vi "Measurement UI.vi"() -> ()   [LabVIEW 2025, in "CAN-LIN Raw Bus Capture UI.lvlib"]
uses:
  CAN-LIN Raw Bus Capture UI.lvlib
  Toggle.ctl
  <vilib>/gRPC/LabVIEW gRPC Library/Shared/grpcId.ctl
  <vilib>/Utility/error.llb/whitespace.ctl
  <vilib>/Utility/error.llb/Trim Whitespace One-Sided.vi
  Get Status.vi
  Create Buffer.vi
  Flush Table.vi
  Destroy Table Buffer.vi
  OOB gRPC Client/OOB gRPC Client.lvlib
  <vilib>/gRPC/LabVIEW gRPC Library/grpc-lvsupport-release.lvlib
panel:
  out "New root item?":bool
  in  "Tree Data":string[][](array[string])
  in  "Mapping done?":bool
  in  "Table map":map{string, i32}(c390)
  in  "XNET Sessions map":map{u32, refnum<k21>}(c390)
  in  "Tags map":map{string, bool}(c390)
  out "Valid DBC file?":bool
  out "Signals in DBC":i32
  out "Frames in DBC":i32
  in  "Frames Map":map{u32, refnum<k21>}(c390)
  in  "Signals Map":map{u32, refnum<k21>[]}(c390)
  in  "Tree and Table":enum32{"Trace window", "Signal table"}(tab)
  out "Frames":string(tree)
  out "Signals":string[][](table)
  in  "HELP":bool
  out "IsRestarting?":bool
  out "Table Buffer":i32
  out "Error (Logic)":string
  out "Status Message":string
  in  "SAVE FORMAT":u16(ring) items=["TDMS", "CSV"]
  out "Connection":bool
  in  "Clear Trace":bool
  in  "Bus Type":string="CAN"
  in  "Lin Interface":string
  in  "Can Interface":string
  in  "PauseResume":bool
  in  "Path":path
  in  "Save":bool
  in  "Filter":string
  in  "SortByID":bool
  out "Status":string
  in  "SETTINGS":enum32{"CAN", "LIN"}(tab)
  in  "Run Mode":enum32{"Normal", "Subordinate"}(ring)
  in  "IO Mode":enum32{"CAN", "CAN FD", "CAN FD + BRS"}(ring)
  in  "FD ISO Mode":enum32{"ISO", "Non ISO", "Legacy ISO"}(ring)
  in  "Baudrate":u32=125000
  in  "FD Baudrate":u32=1000000
  in  "Termination CAN":T1
  in  "INTERFACE NAME CAN":refnum<k21>
  in  "DBC path":path
  in  "Termination LIN":T1
  in  "INTERFACE NAME LIN":refnum<k21>
  out "Buffer Size":i32
  out "OOB gRPC Port":i32
  # "CONFIGURATION"
  # "CONTROL"
  # "DBC INFORMATION"
  # "STATUS"
  # "CAN Settings"
  # "LIN Settings"
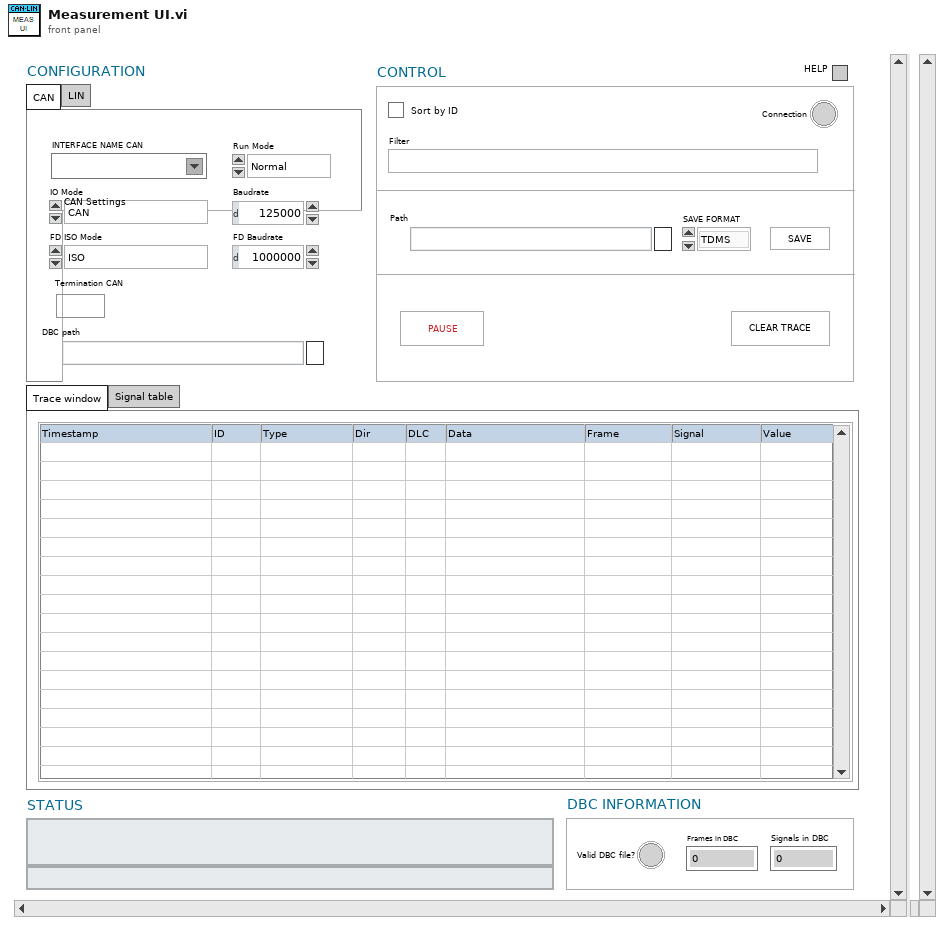
[diagram p1: front panel]
types:
  T1 = typedef "Toggle.ctl" = bool
  T2 = typedef "grpc-lvsupport-release.lvlib/grpcId.ctl" = u64
  T3 = cluster{"Tree and Table":refnum<vi>, "New root item?":refnum<vi>, "Tree Data":refnum<vi>, "Mapping done?":refnum<vi>, "Table map":refnum<vi>, "Tags map":refnum<vi>, "XNET Sessions map":refnum<vi>, "Signals":refnum<vi>, "PauseResume":refnum<vi>, "Clear Trace":refnum<vi>, "Path":refnum<vi>, "SAVE FORMAT":refnum<vi>, "Save":refnum<vi>, "Bus Type":refnum<vi>, "Filter":refnum<vi>, "SortByID":refnum<vi>, "Status Message":refnum<vi>, "Frames":refnum<vi>, "DBC path":refnum<vi>, "Signals Map":refnum<vi>, "Frames Map":refnum<vi>, "Frames in DBC":refnum<vi>, "Signals in DBC":refnum<vi>, "Valid DBC file?":refnum<vi>}
  T4 = typedef "whitespace.ctl" = u16
  T5 = enum32{"Page Enabled", "Page Disabled", "Page Disabled & Grayed"}
  T6 = enum8{"Enabled", "Disabled", "Disabled and Grayed Out"}
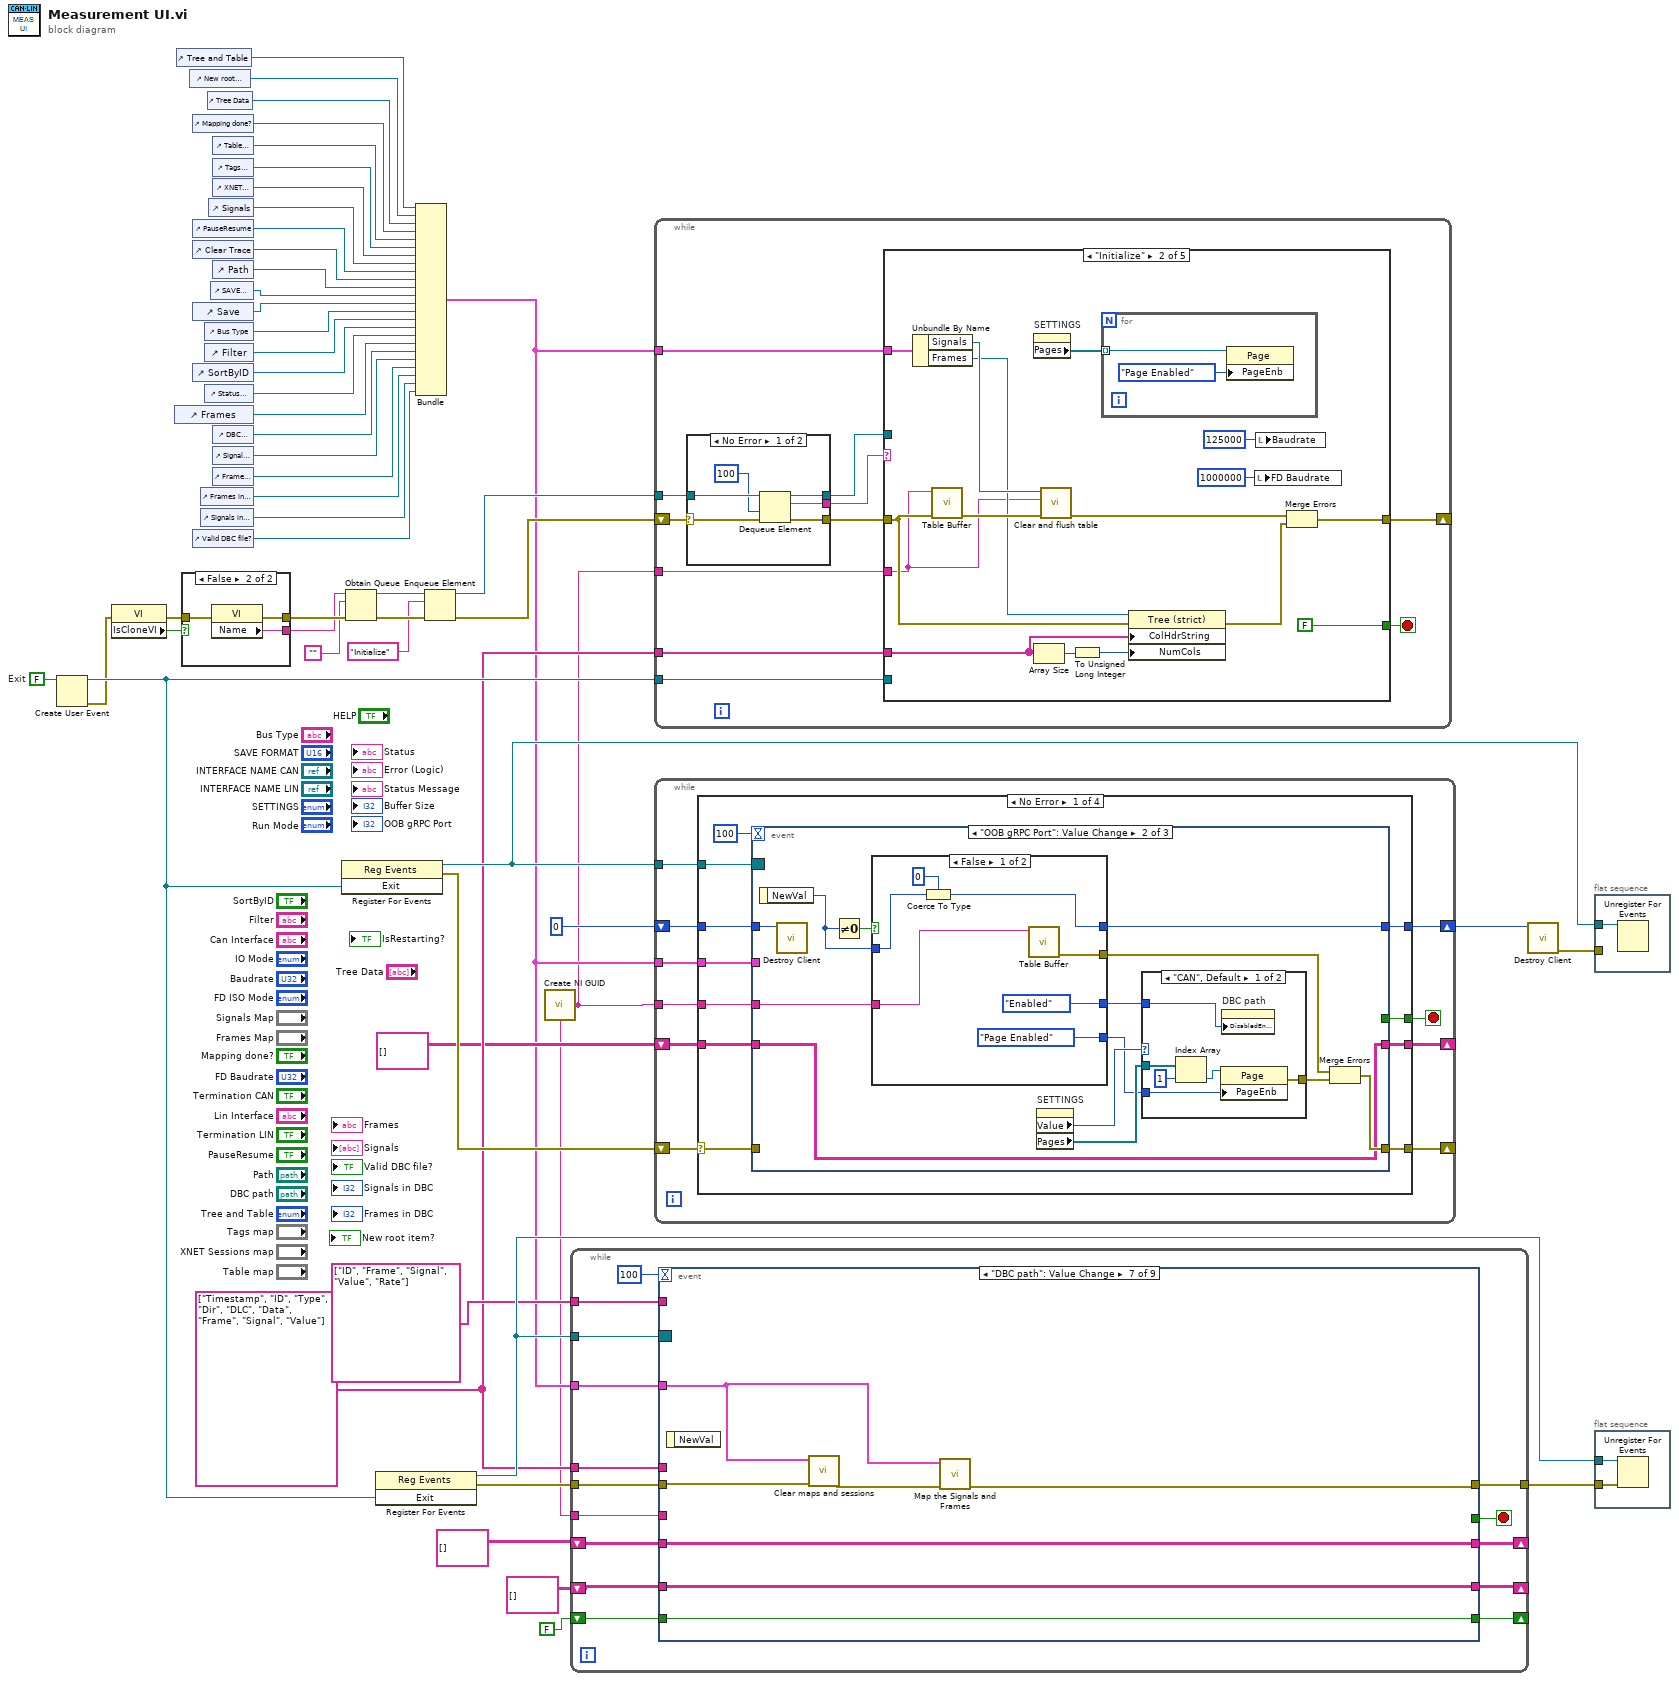
[diagram p0: block diagram]
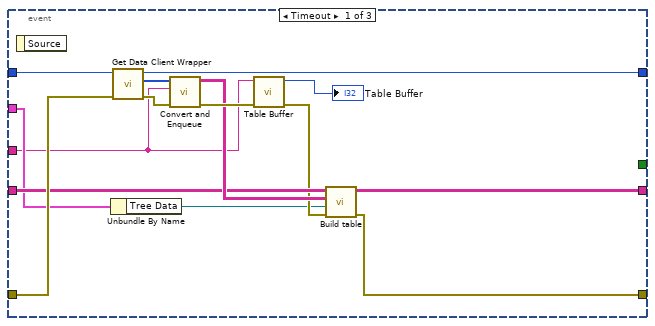
[diagram p2: hidden frame]
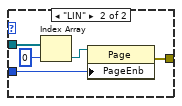
[diagram p3: hidden frame]
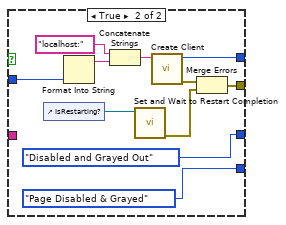
[diagram p4: hidden frame]
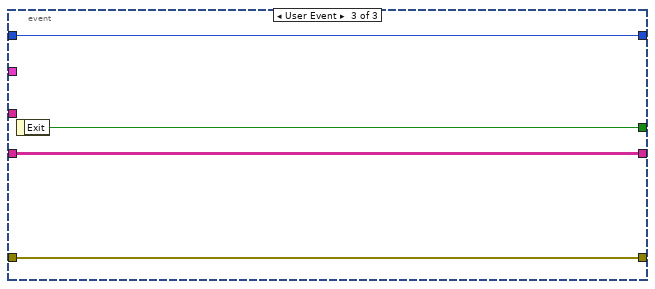
[diagram p5: hidden frame]
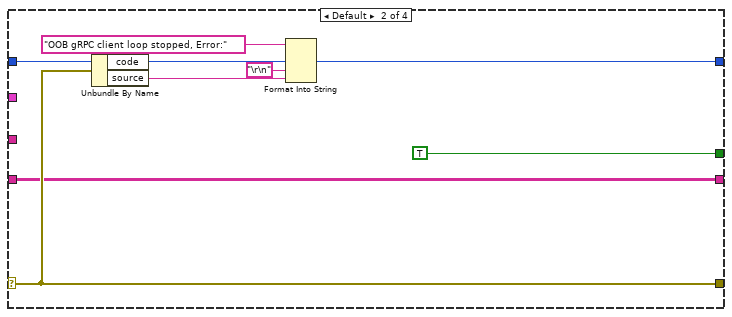
[diagram p6: hidden frame]
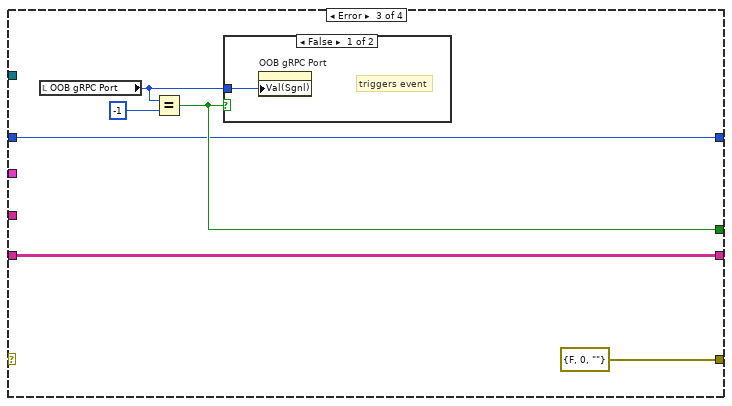
[diagram p7: hidden frame]
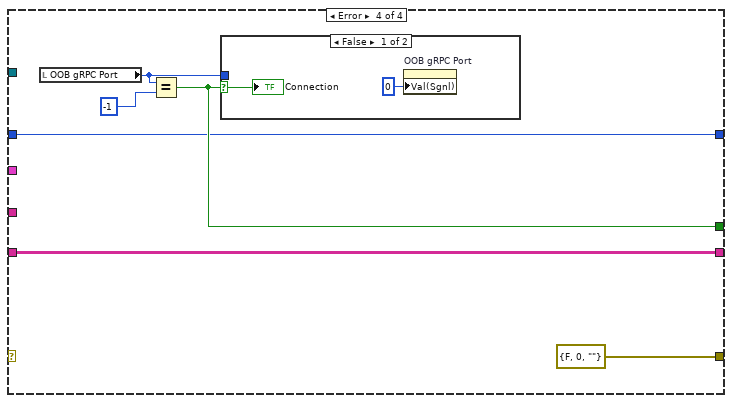
[diagram p9: hidden frame]
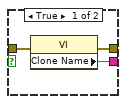
[diagram p11: hidden frame]
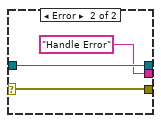
[diagram p12: hidden frame]
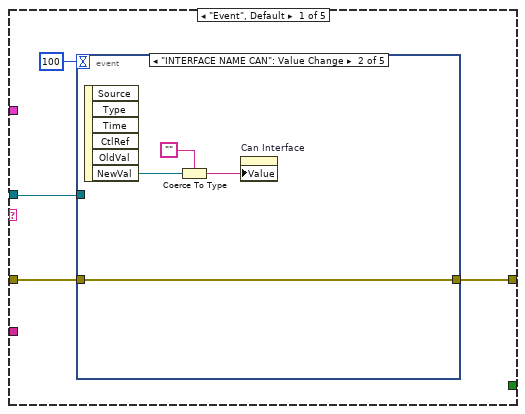
[diagram p13: hidden frame]
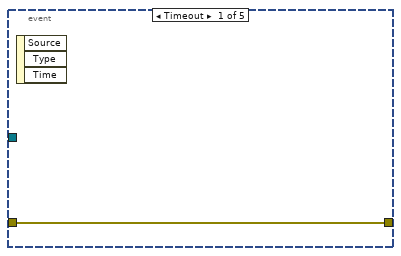
[diagram p14: hidden frame]
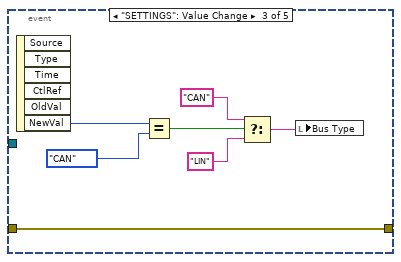
[diagram p15: hidden frame]
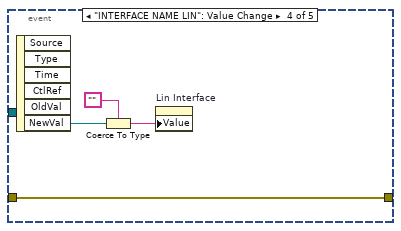
[diagram p16: hidden frame]
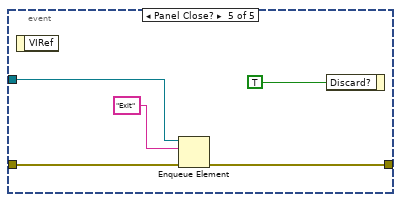
[diagram p17: hidden frame]
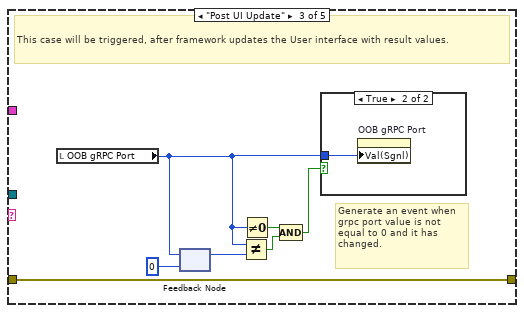
[diagram p18: hidden frame]
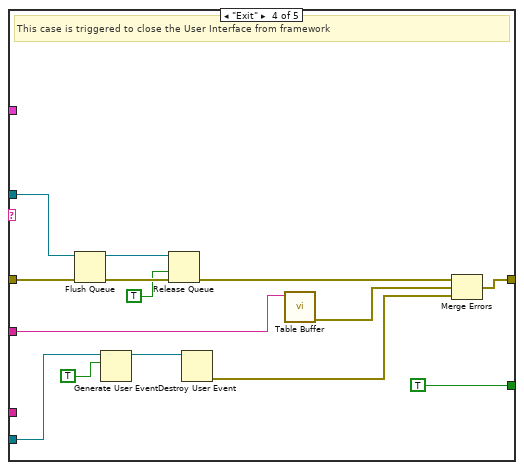
[diagram p20: hidden frame]
diagram:
  w21 = string[] ["Timestamp", "ID", "Type", "Dir", "DLC", "Data", "Frame", "Signal", "Value"] ("Headers")
  w45 = FALSE  # Exit
  n1 = Create User Event(user event datatype=w45) -> (user event=w39:refnum<user-event>, error out=w11:errorcluster)  [unwired: 1 in]
  n2 = property class="VI"(error in=w11) -> (error out=w46:errorcluster, "IsCloneVI"=w47:bool)  [unwired: 1 in, 1 out]
  n3 = control-ref of="Frames"() -> (w25:refnum<vi>)
  n4 = control-ref of="Tree and Table"() -> (w5:refnum<vi>)
  n5 = case shown="False" w47 {
    tunnel: [w56 w59] -> w53
    tunnel: [w55 w58] -> w52
    tunnel: w46 -> [w54 w57]
    frame True {
      n6 = property class="VI"(error in=w54) -> (error out=w56:errorcluster, "Clone Name"=w55:string)  [unwired: 1 in, 1 out]
    }
    frame False {
      n7 = property class="VI"(error in=w57) -> (error out=w59:errorcluster, "Name"=w58:string)  [unwired: 1 in, 1 out]
    }
  }
  n8 = control-ref of="New root item?"() -> (w6:refnum<vi>)
  n9 = control-ref of="Mapping done?"() -> (w9:refnum<vi>)
  n10 = control-ref of="PauseResume"() -> (w29:refnum<vi>)
  n11 = control-ref of="Clear Trace"() -> (w37:refnum<vi>)
  n12 = control-ref of="Save"() -> (w34:refnum<vi>)
  n13 = control-ref of="SortByID"() -> (w32:refnum<vi>)
  n14 = control-ref of="Valid DBC file?"() -> (w17:refnum<vi>)
  n15 = control-ref of="Frames in DBC"() -> (w19:refnum<vi>)
  n16 = control-ref of="Signals in DBC"() -> (w18:refnum<vi>)
  n17 = control-ref of="Bus Type"() -> (w33:refnum<vi>)
  n18 = control-ref of="Filter"() -> (w31:refnum<vi>)
  n19 = control-ref of="Status Message"() -> (w30:refnum<vi>)
  n20 = control-ref of="Tree Data"() -> (w7:refnum<vi>)
  n21 = control-ref of="Signals"() -> (w38:refnum<vi>)
  n22 = control-ref of="SAVE FORMAT"() -> (w35:refnum<vi>)
  n23 = control-ref of="Table map"() -> (w14:refnum<vi>)
  n24 = control-ref of="Tags map"() -> (w16:refnum<vi>)
  n25 = control-ref of="XNET Sessions map"() -> (w15:refnum<vi>)
  n26 = control-ref of="Path"() -> (w36:refnum<vi>)
  n27 = control-ref of="DBC path"() -> (w26:refnum<vi>)
  n28 = control-ref of="Signals Map"() -> (w22:refnum<vi>)
  n29 = control-ref of="Frames Map"() -> (w23:refnum<vi>)
  n30 = register-events(w39) -> (reference out=w41:refnum<event-registration>, error out=w44:errorcluster)  [unwired: 2 in]
  n31 = Obtain Queue(name (unnamed)=w52, element data type="", error in (no error)=w53) -> (queue out=w50:refnum<queue>, error out=w51:errorcluster)  [unwired: 2 in, 1 out]
  n32 = register-events(w39) -> (reference out=w28:refnum<event-registration>, error out=w12:errorcluster)  [unwired: 2 in]
  n33 = Bundle("Tree and Table"=w5, "New root item?"=w6, "Tree Data"=w7, "Mapping done?"=w9, "Table map"=w14, "Tags map"=w16, "XNET Sessions map"=w15, "Signals"=w38, "PauseResume"=w29, "Clear Trace"=w37, "Path"=w36, "SAVE FORMAT"=w35, "Save"=w34, "Bus Type"=w33, "Filter"=w31, "SortByID"=w32, "Status Message"=w30, "Frames"=w25, "DBC path"=w26, "Signals Map"=w22, "Frames Map"=w23, "Frames in DBC"=w19, "Signals in DBC"=w18, "Valid DBC file?"=w17) -> (w4:T3)  [unwired: 1 in]
  n34 = Enqueue Element(queue=w50, element="Initialize", error in (no error)=w51) -> (queue out=w20:refnum<queue>, error out=w13:errorcluster)  [unwired: 1 in, 1 out]
  n35 = call <vilib>:"Create NI GUID.vi"() -> ("NI GUID"=w3:string)
  n36 = while {
    tunnel: w12 -> [w74]
    tunnel: [w69] -> w10
    tunnel: w28 -> [w73]
    tunnel: w4 -> [w70]
    shift-right: [w67] -> _
    shift-left: string[][] [] ("Table Data out") -> [w68]
    tunnel: string[] ["ID", "Frame", "Signal", "Value", "Rate"] ("Signal Table Headers") -> [w66]
    tunnel: w21 -> [w64]
    tunnel: w3 -> [w65]
    shift-right: [w63] -> _
    shift-left: string[][] [] ("Table Data out") -> [w62]
    shift-right: [w60] -> _
    shift-left: FALSE -> [w61]
    stop <- w72 stop-if-true
    n37 = event shown="[6] \"DBC path\": Value Change" {
      selector: w73 -> [_ _ _ _ _ _ _ _ _]
      dyn-events: _ -> [_ _ _ _ _ _ _ _ _]
      timeout: 100 -> [_ _ _ _ _ _ _ _ _]
      tunnel: w74 -> [w99 w114 w128 w169 w204 w215 w283 w291 w295]
      tunnel: [w83 w113 w142 w168 w189 w222 w281 w290 w295] -> w69
      tunnel: [_ _ _ _ _ _ _ _ w296] -> w72
      tunnel: w70 -> [w97 _ w129 w170 w206 w218 w284 _ _]
      tunnel: w68 -> [w94 w112 w136 w167 w201 w217 w280 w289 w294]
      tunnel: [w107 w112 w137 w167 w201 w217 w280 w289 w294] -> w67
      tunnel: w66 -> [w100 _ _ _ w200 _ _ _ _]
      tunnel: w64 -> [w81 _ _ w165 _ w207 _ _ _]
      tunnel: w65 -> [w77 _ _ _ _ _ _ _ _]
      tunnel: w62 -> [w76 w111 w127 w164 w186 w208 w279 w286 w293]
      tunnel: [w76 w109 w125 w164 w186 w213 w279 w286 w293] -> w63
      tunnel: w61 -> [w75 w110 w126 w163 w185 w210 w278 w285 w292]
      tunnel: [w75 w108 w124 w163 w185 w216 w278 w285 w292] -> w60
      event Timeout {
        n38 = event-data() -> ()  [unwired: 1 in, 1 out]
        n39 = Unbundle By Name(w97) -> ("Signals"=w102:refnum<vi>, "Filter"=w84:refnum<vi>, "SortByID"=w104:refnum<vi>, "Table map"=w95:refnum<vi>, "PauseResume"=w96:refnum<vi>)
        n40 = call "Map the Signals and Frames.vi"("error in"=w99, "References"=w97) -> ("error out"=w98:errorcluster)  [unwired: 9 in]
        n41 = call "PauseResume.vi"("error in"=w98, "UI GUID"=w77, "PauseResume Ref"=w96) -> ("error out"=w92:errorcluster, "Data"=w101:string[][])  [unwired: 7 in]
        n42 = property class="VI"(error in=w92) -> (error out=w93:errorcluster, "Panel"=w89:refnum<vi>)  [unwired: 1 in, 1 out]
        n43 = property class="Pnl"(reference=w89, error in=w93, "DeferPanUpdts"=TRUE ("Defer Panel Updates")) -> (error out=w91:errorcluster)  [unwired: 1 out]
        n44 = call "Update Trace Tree.vi"("References"=w97, "error in"=w91, "Headers"=w81, "Data IN"=w101) -> ("error out"=w85:errorcluster, "Signals"=w88:string[][])  [unwired: 6 in]
        n45 = call "Update Table.vi"("Table map"=w95, "error in"=w85, "New Data in"=w88, "Table Data in"=w94) -> ("error out"=w82:errorcluster, "Table Data out"=w107:string[][])  [unwired: 6 in]
        n46 = property class="VI"(error in=w82) -> (error out=w80:errorcluster, "Panel"=w86:refnum<vi>)  [unwired: 1 in, 1 out]
        n47 = property class="Pnl"(reference=w86, "DeferPanUpdts"=FALSE ("Defer Panel Updates")) -> (error out=w79:errorcluster)  [unwired: 1 in, 1 out]
        n48 = Empty Array?(array=w88) -> (empty?=w103:bool)
        n49 = Merge Errors(w79, w80) -> (w78:errorcluster)
        n50 = call "SortByID.vi"("Headers"=w100, "Trace"=w102, "error in"=w78, "Unsorted Data"=w107, "SortByID"=w104, "Filter"=w84) -> ("error out"=w106:errorcluster, "Table Control"=w105:string[][])  [unwired: 4 in]
        n51 = call "Programatic Scroll.vi"("error in"=w106, "Pause? (F)"=w103, "Table Ref"=w102, "Trace"=w105) -> ("error out"=w83:errorcluster)  [unwired: 7 in]
      }
      event "Clear Trace": Value Change {
        # "Run when restarting or then button is pressed down."
        n52 = event-data() -> ("NewVal"=w115:bool)  [unwired: 1 in]
        n53 = case shown="False" w115 {
          tunnel: w114 -> [w120 w123]
          tunnel: [w118 w123] -> w113
          tunnel: w111 -> [w117 _]
          tunnel: w110 -> [w116 _]
          tunnel: [w117 string[][] [] ("Table Data out")] -> w109
          tunnel: [w116 FALSE] -> w108
          frame False {
            n54 = property on="IsRestarting?" class="Bool (strict)"(error in=w120, "Val(Sgnl)"=FALSE ("Value (Signaling)")) -> (error out=w118:errorcluster)  [unwired: 1 in, 1 out]
          }
          frame True {
          }
        }
      }
      event "IsRestarting?": Value Change {
        n55 = event-data() -> ("NewVal"=w131:bool)  [unwired: 1 in]
        n56 = Unbundle By Name(w129) -> ("Table map"=w132:refnum<vi>, "Tags map"=w133:refnum<vi>, "Frames"=w134:refnum<vi>, "Status Message"=w138:refnum<vi>, "Signals"=w140:refnum<vi>)
        n57 = case shown="False" w131 {
          tunnel: w129 -> [_ w150]
          tunnel: w128 -> [w145 w149]
          tunnel: [w145 w148] -> w130
          tunnel: w127 -> [w144 _]
          tunnel: w126 -> [w143 _]
          tunnel: [w144 string[][] [] ("Table Data out")] -> w125
          tunnel: [w143 FALSE] -> w124
          frame False {
          }
          frame True {
            n58 = call "Clear maps and sessions.vi"("error in"=w149, "References"=w150) -> ("error out"=w148:errorcluster)  [unwired: 9 in]
          }
        }
        n59 = Not(x=w131) -> (.not. x?=w141:bool)
        n60 = call "Clear Table.vi"("error in"=w130, "Confirm? (F)"=w141, "Table in"=w140) -> ("error out"=w139:errorcluster, "T button?"=w135:bool)  [unwired: 7 in]
        n61 = case shown="True" w135 {
          tunnel: [w152 w161] -> w142
          tunnel: w139 -> [w152 w159]
          tunnel: w138 -> [_ w158]
          tunnel: [w151 string[][] [] ("Table Data out")] -> w137
          tunnel: w136 -> [w151 _]
          tunnel: w134 -> [_ w155]
          tunnel: w133 -> [_ w154]
          tunnel: w132 -> [_ w153]
          frame False {
          }
          frame True {
            # "Reset Table when necessary"
            n62 = invoke class="Map (strict)" method="Reinit To Default"(reference=w153) -> ()  [unwired: 2 in, 3 out]
            n63 = invoke class="Map (strict)" method="Reinit To Default"(reference=w154) -> ()  [unwired: 2 in, 3 out]
            n64 = property class="Str"(reference=w158, error in=w159, "Value"="") -> (error out=w160:errorcluster)  [unwired: 1 out]
            n65 = property on="IsRestarting?" class="Bool (strict)"(error in=w160, "Value"=FALSE ("IsRestarting?")) -> (error out=w161:errorcluster)  [unwired: 1 in, 1 out]
            n66 = invoke on="Invoke Node" class="Tree (strict)" method="Edit Tree Items.Delete"(reference=w155) -> ()  [unwired: 4 in, 5 out]
          }
        }
      }
      event "Save": Value Change {
        n67 = event-data() -> ("NewVal"=w166:bool)  [unwired: 1 in]
        n68 = case shown="False" w166 {
          tunnel: w170 -> [_ w184]
          tunnel: w169 -> [w171 w180]
          tunnel: [w171 w178] -> w168
          tunnel: w165 -> [_ w176]
          frame True {
          }
          frame False {
            n69 = Unbundle By Name(w184) -> ("DBC path"=w173:refnum<vi>, "Status Message"=w175:refnum<vi>, "Path"=w183:refnum<vi>, "SAVE FORMAT"=w182:refnum<vi>, "Bus Type"=w181:refnum<vi>, "Tree Data"=w172:refnum<vi>, "Frames"=w174:refnum<vi>)
            n70 = call "Save CAN data.vi"("Frames"=w174, "DBC path"=w173, "Tree Data"=w172, "Headers"=w176, "error in"=w180, "Bus Type"=w181, "Format"=w182, "Path"=w183) -> ("error out"=w179:errorcluster, "Status"=w177:string)  [unwired: 2 in]
            n71 = property class="Str"(reference=w175, error in=w179, "Value"=w177) -> (error out=w178:errorcluster)  [unwired: 1 out]
          }
        }
      }
      event "SortByID": Value Change {
        # "This currently only checks the sorting value change,\nmigth need to check the  Filter Value Change too."
        n72 = event-data() -> ()  [unwired: 1 in, 1 out]
        n73 = Unbundle By Name(w206) -> ("Tags map"=w198:refnum<vi>, "Frames"=w199:refnum<vi>, "Signals"=w203:refnum<vi>, "Filter"=w202:refnum<vi>, "SortByID"=w205:refnum<vi>)
        n74 = call "SortByID.vi"("Headers"=w200, "Trace"=w203, "error in"=w204, "Unsorted Data"=w201, "SortByID"=w205, "Filter"=w202) -> ("error out"=w195:errorcluster)  [unwired: 4 in, 1 out]
        n75 = property class="VI"(error in=w195) -> (error out=w197:errorcluster, "Panel"=w188:refnum<vi>)  [unwired: 1 in, 1 out]
        n76 = property class="Pnl"(reference=w188, error in=w197, "DeferPanUpdts"=TRUE ("Defer Panel Updates")) -> (error out=w194:errorcluster)  [unwired: 1 out]
        n77 = call "Order tree.vi"("Tags map"=w198, "error in"=w194, "TreeControl in"=w199) -> ("error out"=w192:errorcluster)  [unwired: 8 in]
        n78 = property class="VI"(error in=w192) -> (error out=w190:errorcluster, "Panel"=w187:refnum<vi>)  [unwired: 1 in, 1 out]
        n79 = property class="Pnl"(reference=w187, "DeferPanUpdts"=FALSE ("Defer Panel Updates")) -> (error out=w191:errorcluster)  [unwired: 1 in, 1 out]
        n80 = Merge Errors(w190, w191) -> (w189:errorcluster)
      }
      event "Filter": Value Change {
        w220 = T4 0 items=["both", "start of string", "end of string"] ("location (both)")
        n81 = event-data() -> ("NewVal"=w221:string)  [unwired: 1 in]
        n82 = Unbundle By Name(w218) -> ("Frames"=w214:refnum<vi>, "Tags map"=w212:refnum<vi>, "Filter"=w211:refnum<vi>)
        n83 = call <vilib>:"Trim Whitespace.vi"("string"=w221, "location (both)"=w220) -> ("trimmed string"=w219:string)
        n84 = Empty String/Path?(string/path=w219) -> (empty?=w209:bool)
        n85 = case shown="True" w210 {
          tunnel: [w231 w246] -> w222
          tunnel: w207 -> [w230 w247]
          tunnel: [w229 w244] -> w216
          tunnel: w215 -> [w228 w252]
          tunnel: w214 -> [w227 w251]
          tunnel: [w226 w245] -> w213
          tunnel: w212 -> [w225 w250]
          tunnel: w211 -> [w224 w248]
          tunnel: w209 -> [w223 w253]
          tunnel: w208 -> [_ w249]
          frame False {
            n86 = case shown="False" w223 {
              tunnel: [w233 w243] -> w231
              tunnel: w227 -> [w234 _]
              tunnel: w228 -> [w239 w243]
              tunnel: w230 -> [w232 _]
              tunnel: [TRUE FALSE] -> w229
              tunnel: [w238 string[][] [] ("Array")] -> w226
              tunnel: w225 -> [w235 _]
              tunnel: w224 -> [w236 _]
              frame False {
                n87 = call "Get Tree Data.vi"("error in"=w239, "Tree ref"=w234) -> ("error out"=w237:errorcluster, "Array"=w238:string[][])  [unwired: 8 in]
                n88 = call "Filter Tree.vi"("Headers"=w232, "error in"=w237, "Tags map"=w235, "Frames"=w234, "Filter"=w236) -> ("error out"=w233:errorcluster)  [unwired: 6 in]
              }
              frame True {
              }
            }
          }
          frame True {
            n89 = case shown="True" w253 {
              tunnel: w252 -> [w266 w276]
              tunnel: w251 -> [w265 w277]
              tunnel: w250 -> [w264 w275]
              tunnel: w249 -> [w254 w270]
              tunnel: w248 -> [w261 _]
              tunnel: w247 -> [w257 _]
              tunnel: [w256 w267] -> w246
              tunnel: [w254 string[][] [] ("Array")] -> w245
              tunnel: [TRUE FALSE] -> w244
              frame False {
                n90 = invoke class="Tree (strict)" method="Edit Tree Items.Delete"(reference=w265, error in=w266) -> (reference out=w260:refnum<vi>, error out=w263:errorcluster)  [unwired: 3 in, 3 out]
                n91 = invoke class="Map (strict)" method="Reinit To Default"(reference=w264, error in=w263) -> (reference out=w259:refnum<vi>, error out=w262:errorcluster)  [unwired: 1 in, 1 out]
                n92 = call "Re-Populate Tree.vi"("error in"=w262, "Tags map"=w259, "Data in"=w254, "TreeControl in"=w260) -> ("error out"=w258:errorcluster)  [unwired: 7 in]
                n93 = call "Filter Tree.vi"("Headers"=w257, "error in"=w258, "Tags map"=w259, "Frames"=w260, "Filter"=w261) -> ("error out"=w256:errorcluster)  [unwired: 6 in]
              }
              frame True {
                n94 = invoke class="Tree (strict)" method="Edit Tree Items.Delete"(reference=w277, error in=w276) -> (reference out=w273:refnum<vi>, error out=w274:errorcluster)  [unwired: 3 in, 3 out]
                n95 = invoke class="Map (strict)" method="Reinit To Default"(reference=w275, error in=w274) -> (reference out=w272:refnum<vi>, error out=w271:errorcluster)  [unwired: 1 in, 1 out]
                n96 = call "Re-Populate Tree.vi"("error in"=w271, "Tags map"=w272, "Data in"=w270, "TreeControl in"=w273) -> ("error out"=w267:errorcluster)  [unwired: 7 in]
              }
            }
          }
        }
      }
      event "DBC path": Value Change {
        n97 = event-data() -> ()  [unwired: 1 in, 1 out]
        n98 = call "Clear maps and sessions.vi"("error in"=w283, "References"=w284) -> ("error out"=w282:errorcluster)  [unwired: 9 in]
        n99 = call "Map the Signals and Frames.vi"("error in"=w282, "References"=w284) -> ("error out"=w281:errorcluster)  [unwired: 9 in]
      }
      event "HELP": Value Change {
        n100 = event-data() -> ("NewVal"=w288:bool)  [unwired: 1 in]
        n101 = call "Open Help PDF.vi"("error in"=w291, "NewVal"=w288, "Path after documentation"=path "CAN-LIN Raw Bus Capture.pdf") -> ("error out"=w290:errorcluster)  [unwired: 8 in]
      }
      event User Event {
        n102 = event-data() -> ("Exit"=w296:bool)  [unwired: 1 in]
      }
    }
  }
  n103 = while {
    shift-right: [w302] -> _
    shift-left: w13 -> [w307]
    tunnel: w20 -> [w305]
    tunnel: w39 -> [w300]
    tunnel: w4 -> [w299]
    tunnel: w21 -> [w298]
    tunnel: w3 -> [w297]
    stop <- w301 stop-if-true
    n104 = case shown="No Error" w307 {
      selector: w307 -> [w313 w316]
      tunnel: [w312 w316] -> w306
      tunnel: w305 -> [w311 w315]
      tunnel: [w310 w315] -> w304
      tunnel: [w309 "Handle Error"] -> w303
      frame No Error {
        n105 = Dequeue Element(queue=w311, timeout in ms (-1)=100, error in (no error)=w313) -> (queue out=w310:refnum<queue>, element=w309:string, error out=w312:errorcluster)  [unwired: 1 out]
      }
      frame Error {
      }
    }
    n106 = case shown="\"Initialize\"" w303 {
      tunnel: w306 -> [w319 w345 w360 w381 w386]
      tunnel: w304 -> [w318 _ _ w379 w385]
      tunnel: [w320 w348 w360 w370 w386] -> w302
      tunnel: [_ FALSE _ TRUE _] -> w301
      tunnel: w300 -> [_ _ _ w373 _]
      tunnel: w299 -> [_ w343 _ _ _]
      tunnel: w298 -> [_ w344 _ _ _]
      tunnel: w297 -> [_ w342 _ w368 _]
      frame "Event", Default {
        n107 = event shown="[1] \"INTERFACE NAME CAN\": Value Change" {
          selector: _ -> [_ _ _ _ _]
          dyn-events: _ -> [_ _ _ _ _]
          timeout: 100 -> [_ _ _ _ _]
          tunnel: [w321 w325 w327 w336 w340] -> w320
          tunnel: w319 -> [w321 w325 w327 w336 w341]
          tunnel: w318 -> [_ _ _ _ w339]
          event Timeout {
            n108 = event-data() -> ()  [unwired: 1 in, 3 out]
          }
          event "INTERFACE NAME CAN": Value Change {
            n109 = event-data() -> ("NewVal"=w323:refnum<k21>)  [unwired: 1 in, 5 out]
            n110 = Coerce To Type(0:w323, 1:"") -> (2:w322:string)
            n111 = property on="Can Interface" class="Str"("Value"=w322) -> ()  [unwired: 2 in, 2 out]
          }
          event "SETTINGS": Value Change {
            n112 = event-data() -> ("NewVal"=w332:enum32{"CAN", "LIN"})  [unwired: 1 in, 5 out]
            n113 = Equal?(x=w332, y=enum32{"CAN", "LIN"}."CAN") -> (x = y?=w330:bool)
            n114 = Select(t="CAN", s=w330, f="LIN") -> (s? t:f=w326:string)
            n115 = local write "Bus Type"(w326) -> ()
          }
          event "INTERFACE NAME LIN": Value Change {
            n116 = event-data() -> ("NewVal"=w333:refnum<k21>)  [unwired: 1 in, 5 out]
            n117 = Coerce To Type(0:w333, 1:"") -> (2:w334:string)
            n118 = property on="Lin Interface" class="Str"("Value"=w334) -> ()  [unwired: 2 in, 2 out]
          }
          event Panel Close? {
            n119 = event-data() -> ()  [unwired: 1 in, 1 out]
            n120 = Enqueue Element(queue=w339, element="Exit", error in (no error)=w341) -> (error out=w340:errorcluster)  [unwired: 1 in, 2 out]
            n121 = event-data("Discard?"=TRUE) -> ()  [unwired: 1 in, 1 out]
          }
        }
      }
      frame "Initialize" {
        n122 = Unbundle By Name(w343) -> ("Signals"=w354:refnum<vi>, "Frames"=w349:refnum<vi>)
        n123 = call-poly "Table Buffer.vi"("error in (no error)"=w345, "UI GUID"=w342) -> ("error out"=w352:errorcluster)  [unwired: 9 in]
        n124 = property on="SETTINGS" class="TabCtl (strict)"() -> ("Pages"=w353:refnum<vi>[])  [unwired: 2 in, 2 out]
        n125 = Array Size(array=w344) -> (size(s)=w350:i32)
        n126 = call "Clear and flush table.vi"("error in"=w352, "UI GUID"=w342, "Trace"=w354) -> ("error out"=w347:errorcluster)  [unwired: 8 in]
        n127 = To Unsigned Long Integer(number=w350) -> (unsigned 32bit integer=w351:u32)
        n128 = for {
          tunnel: w353 -> [w359] mode=indexing
          n129 = property class="Page"(reference=w359, "PageEnb"=T5."Page Enabled" ("Page Enabled State")) -> ()  [unwired: 1 in, 2 out]
        }
        n130 = property on="Property Node" class="Tree (strict)"(reference=w349, error in=w345, "ColHdrString"=w344, "NumCols"=w351) -> (error out=w346:errorcluster)  [unwired: 1 out]
        n131 = local write "FD Baudrate"(u32 1000000 ("FD Baudrate")) -> ()
        n132 = local write "Baudrate"(u32 125000 ("Baudrate")) -> ()
        n133 = Merge Errors(w347, w346) -> (w348:errorcluster)
      }
      frame "Post UI Update" {
        # "Generate an event when grpc port value is not equal to 0 and it has changed."
        # "This case will be triggered, after framework updates the User interface with result values."
        n134 = local read "OOB gRPC Port"() -> (w363:i32)
        n135 = feedback #1(0 ("OOB gRPC Port")) -> (w362:i32)
        n136 = feedback-in #1(w363) -> ()
        n137 = Not Equal?(x=w363, y=w362) -> (x != y?=w364:bool)
        n138 = Not Equal To 0?(x=w363) -> (x != 0?=w365:bool)
        n139 = Compound Arithmetic op=AND(w365, w364) -> (w361:bool)
        n140 = case shown="True" w361 {
          tunnel: w363 -> [_ w367]
          frame False {
          }
          frame True {
            n141 = property on="OOB gRPC Port" class="DigNum (strict)"("Val(Sgnl)"=w367) -> ()  [unwired: 2 in, 2 out]
          }
        }
      }
      frame "Exit" {
        # "This case is triggered to close the User Interface from framework"
        n142 = Flush Queue(queue=w379, error in (no error)=w381) -> (queue out=w378:refnum<queue>, error out=w377:errorcluster)  [unwired: 1 out]
        n143 = Generate User Event(user event=w373, event data cluster=TRUE ("event data")) -> (user event out=w375:refnum<user-event>)  [unwired: 2 in, 1 out]
        n144 = Release Queue(queue=w378, force destroy? (F)=TRUE, error in (no error)=w377) -> (error out=w369:errorcluster)  [unwired: 2 out]
        n145 = Destroy User Event(user event=w375) -> (error out=w372:errorcluster)  [unwired: 1 in]
        n146 = call-poly "Table Buffer.vi"("UI GUID"=w368) -> ("error out"=w371:errorcluster)  [unwired: 10 in]
        n147 = Merge Errors(w369, w371, w372) -> (w370:errorcluster)
      }
      frame "Handle Error" {
        w384 = "UI main loop stopped, Error: %d - %s" ("format string")
        n148 = Unbundle By Name(w386) -> ("code"=w387:i32, "source"=w382:string)
        n149 = case shown="Default" w386 {
          selector: w386 -> [w388 w393]
          tunnel: [w388 w392] -> _
          tunnel: w385 -> [_ w389]
          frame No Error {
          }
          frame Default {
            n150 = call <vilib>:"Clear Errors.vi"("error in (no error)"=w393) -> ("error out"=w391:errorcluster)  [unwired: 5 in, 1 out]
            n151 = Enqueue Element At Opposite End(queue=w389, element="Exit", error in (no error)=w391) -> (error out=w392:errorcluster)  [unwired: 1 in, 2 out]
          }
        }
        n152 = Format Into String(format string=w384, initial string=w384, w387, w382) -> (resulting string=w383:string)  [unwired: 1 in, 1 out]
        n153 = local write "Status Message"(w383) -> ()
      }
    }
  }
  n154 = while {
    tunnel: w41 -> [w400]
    shift-right: [w401] -> _
    shift-left: w44 -> [w403]
    shift-right: [w398] -> w42
    shift-left: T2 0 ("gRPC ID out") -> [w399]
    tunnel: w4 -> [w397]
    shift-right: [w395] -> _
    shift-left: string[][] [] ("Table Data in") -> [w396]
    tunnel: w3 -> [w394]
    stop <- w402 stop-if-true
    n155 = case shown="No Error" w403 {
      selector: w403 -> [w412 w477 _ _]
      tunnel: [w409 TRUE w487 w494] -> w402
      tunnel: [w413 w477 errorcluster {"status"=FALSE, "code"=0, "source"=""} ("error IO") errorcluster {"status"=FALSE, "code"=0, "source"=""} ("error IO")] -> w401
      tunnel: w400 -> [w414 _ _ _]
      tunnel: w399 -> [w411 w482 w486 w493]
      tunnel: [w410 w482 w486 w493] -> w398
      tunnel: w397 -> [w407 _ _ _]
      tunnel: w396 -> [w406 w476 w484 w491]
      tunnel: [w405 w476 w484 w491] -> w395
      tunnel: w394 -> [w404 _ _ _]
      frame No Error {
        n156 = event shown="[1] \"OOB gRPC Port\": Value Change" {
          selector: w414 -> [_ _ _]
          dyn-events: _ -> [_ _ _]
          timeout: 100 -> [_ _ _]
          tunnel: [w419 w433 w473] -> w413
          tunnel: w412 -> [w423 _ w473]
          tunnel: w411 -> [w424 w442 w474]
          tunnel: [w429 w441 w474] -> w410
          tunnel: [_ _ w475] -> w409
          tunnel: w407 -> [w417 _ _]
          tunnel: w406 -> [w421 w431 w472]
          tunnel: [w418 w431 w472] -> w405
          tunnel: w404 -> [w415 w430 _]
          event Timeout {
            n157 = event-data() -> ()  [unwired: 1 in, 1 out]
            n158 = Unbundle By Name(w417) -> ("Tree Data"=w416:refnum<vi>)
            n159 = call "Get Data Client Wrapper.vi"("error in"=w423, "gRPC ID in"=w424) -> ("error out"=w428:errorcluster, "Payload"=w427:u8[], "gRPC ID out"=w429:T2)  [unwired: 7 in]
            n160 = call "Convert and Enqueue.vi"("error in"=w428, "UI GUID"=w415, "Data"=w427) -> ("error out"=w426:errorcluster, "Table Data"=w422:string[][])  [unwired: 7 in]
            n161 = call-poly "Table Buffer.vi"("error in"=w426, "UI GUID"=w415) -> ("error out"=w420:errorcluster, "Messages"=→"Table Buffer":i32)  [unwired: 8 in]
            n162 = call "Build table.vi"("error in"=w420, "Tree Data"=w416, "New Data in"=w422, "Tree Data in"=w421) -> ("error out"=w419:errorcluster, "Tree Data out"=w418:string[][])  [unwired: 6 in]
          }
          event "OOB gRPC Port": Value Change {
            n163 = event-data() -> ("NewVal"=w439:i32)  [unwired: 1 in]
            n164 = call "Destroy Client.vi"("gRPC ID"=w442) -> ()  [unwired: 10 in, 1 out]
            n165 = Not Equal To 0?(x=w439) -> (x != 0?=w440:bool)
            n166 = case shown="False" w440 {
              tunnel: [w456 w464] -> w434
              tunnel: w439 -> [w459 w468]
              tunnel: [w457 w467] -> w441
              tunnel: [T5."Page Enabled" ("Page Enabled State") T5."Page Disabled & Grayed" ("Page Enabled State")] -> w436
              tunnel: [T6."Enabled" ("DisabledEnum") T6."Disabled and Grayed Out" ("DisabledEnum")] -> w432
              tunnel: w430 -> [w454 _]
              frame False {
                n167 = Coerce To Type(0:w459, 1:T2 0 ("gRPC ID Out")) -> (2:w457:T2)
                n168 = call-poly "Table Buffer.vi"("UI GUID"=w454) -> ("error out"=w456:errorcluster)  [unwired: 10 in]
              }
              frame True {
                n169 = control-ref of="IsRestarting?"() -> (w462:refnum<vi>)
                n170 = Format Into String(w468) -> (resulting string=w471:string)  [unwired: 3 in, 1 out]
                n171 = Concatenate Strings("localhost:" ("string"), w471) -> (w469:string)
                n172 = call "Set and Wait to Restart Completion.vi"("Bool Ref"=w462) -> ("error out"=w463:errorcluster)  [unwired: 10 in]
                n173 = call "Create Client.vi"("address"=w469) -> ("error out"=w465:errorcluster, "gRPC ID Out"=w467:T2)  [unwired: 9 in]
                n174 = Merge Errors(w465, w463) -> (w464:errorcluster)
              }
            }
            n175 = property on="SETTINGS" class="TabCtl (strict)"() -> ("Value"=w438:enum32{"CAN", "LIN"}, "Pages"=w437:refnum<vi>[])  [unwired: 2 in, 2 out]
            n176 = case shown="\"CAN\", Default" w438 {
              tunnel: w437 -> [w448 w453]
              tunnel: w436 -> [w445 w451]
              tunnel: [w444 w449] -> w435
              tunnel: w432 -> [w443 _]
              frame "CAN", Default {
                n177 = Index Array(array=w448, index=1) -> (element=w446:refnum<vi>)
                n178 = property class="Page"(reference=w446, "PageEnb"=w445) -> (error out=w444:errorcluster)  [unwired: 1 in, 1 out]
                n179 = property on="DBC path" class="Path"("DisabledEnum"=w443) -> ()  [unwired: 2 in, 2 out]
              }
              frame "LIN" {
                n180 = Index Array(array=w453, index=0) -> (element=w452:refnum<vi>)
                n181 = property class="Page"(reference=w452, "PageEnb"=w451) -> (error out=w449:errorcluster)  [unwired: 1 in, 1 out]
              }
            }
            n182 = Merge Errors(w434, w435) -> (w433:errorcluster)
          }
          event User Event {
            n183 = event-data() -> ("Exit"=w475:bool)  [unwired: 1 in]
          }
        }
      }
      frame Default {
        n184 = Unbundle By Name(w477) -> ("code"=w481:i32, "source"=w480:string)
        n185 = Format Into String(initial string="OOB gRPC client loop stopped, Error:" ("format string"), w481, "\r\n", w480) -> ()  [unwired: 2 in, 2 out]
      }
      frame Error {
        n186 = local read "OOB gRPC Port"() -> (w489:i32)
        n187 = Equal?(x=w489, y=-1 ("x")) -> (x = y?=w487:bool)
        n188 = case shown="False" w487 {
          tunnel: w489 -> [w490 _]
          frame False {
            # "triggers event"
            n189 = property on="OOB gRPC Port" class="DigNum (strict)"("Val(Sgnl)"=w490) -> ()  [unwired: 2 in, 2 out]
          }
          frame True {
          }
        }
      }
      frame Error {
        n190 = local read "OOB gRPC Port"() -> (w496:i32)
        n191 = Equal?(x=w496, y=-1 ("x")) -> (x = y?=w494:bool)
        n192 = case shown="False" w494 {
          selector: w494 -> [w497 _]
          tunnel: w496 -> [_ _]
          frame False {
            n193 = property on="OOB gRPC Port" class="DigNum (strict)"("Val(Sgnl)"=0 ("Value (Signaling)")) -> ()  [unwired: 2 in, 2 out]
            "Connection" <- w497
          }
          frame True {
          }
        }
      }
    }
  }
  n194 = call "Destroy Client.vi"("gRPC ID"=w42) -> ("error out"=w43:errorcluster)  [unwired: 10 in]
  n195 = flat-sequence {
    tunnel: w41 -> [w499]
    tunnel: w43 -> [_]
    frame #0 {
      n196 = Unregister For Events(event registration refnum=w499) -> ()  [unwired: 1 in, 1 out]
    }
  }
  n197 = flat-sequence {
    tunnel: w28 -> [w501]
    tunnel: w10 -> [w500]
    frame #0 {
      n198 = Unregister For Events(event registration refnum=w501, error in=w500) -> ()  [unwired: 1 out]
    }
  }
